vi "UMLEditor Main.vi"(1 "StartProject":string, 3 "StartTarget":string) -> ()   [LabVIEW 2020] (continued)
                        n383 = case shown="1.." w1168 {
                          tunnel: w1174 -> [w1175 w1184]
                          tunnel: [w1176 w1181] -> w1173
                          tunnel: [w1175 w1190] -> w1172
                          tunnel: w1171 -> [w1176 w1189]
                          tunnel: w1170 -> [_ w1188]
                          tunnel: w1169 -> [_ w1187]
                          tunnel: w1167 -> [_ w1183]
                          tunnel: w1166 -> [_ w1180]
                          frame 0, Default {
                          }
                          frame 1.. {
                            n384 = Index Array(array=w1187) -> (element=w1193:refnum<class "AbstractNode.lvclass">)  [unwired: 1 in]
                            n385 = Equal?(x=w1188, y=UMLEditor_HotSpotType."Collaps") -> (x = y?=w1194:bool)
                            n386 = call-dynamic "Collaps.vi"("reference in"=w1193, "Collaps"=w1194, "error in (no error)"=w1189) -> ("reference out"=w1179:refnum<class "AbstractNode.lvclass">, "error out"=w1192:errorcluster)  [unwired: 15 in]
                            n387 = Bundle By Name(cluster=w1184, "newSelected"=FALSE ("HotSpotCursor"), "state"=UMLEditor_statesType."Repaint", "lastMousePoint"=w1183) -> (w1185:T5)
                            n388 = Build Array(w1179) -> (w1178:refnum<class "AbstractNode.lvclass">[])
                            n389 = call <resource>:"UMLEditor setDiagramInfo.vi"("error in (no error)"=w1192, "localVariablesIn"=w1185, "action"=enum16{"Name/Dir", "Unsaved", "Saved"}."Unsaved") -> ("localVariablesOut"=w1190:T5, "error out"=w1182:errorcluster)  [unwired: 2 in, 13 out]
                            n390 = call-dynamic "layout.vi"("reference"=w1180, "LayoutNodes(Empty=All)"=w1178, "error in (no error)"=w1182) -> ("error out"=w1181:errorcluster)  [unwired: 15 in, 1 out]
                          }
                        }
                      }
                    }
                  }
                }
              }
              frame True {
              }
            }
            n391 = Bundle By Name(cluster=w899, "ShiftDown"=w880, "CtrlDown"=w880, "butDwn"=w880, "rubberBandStart"=w905, "dragStartPoint"=w905, "dragStartBounds"=T10 {"x"=nan, "y"=nan, "width"=nan, "height"=nan}) -> (w876:T5)
          }
          event "Picture": Mouse Wheel {
            n392 = event-data() -> ("Delta"=w1199:i32, "Orientation"=w1203:enum16{"Horizontal", "Vertical"}, "PlatMods"=w1205:T45)  [unwired: 3 out]
            n393 = Unbundle By Name(w1206) -> ("NodesBounds"=w1207:T10)
            n394 = Unbundle By Name(w1205) -> ("Ctrl"=w1204:bool)
            n395 = Multiply(x=w1199, y=25) -> (x*y=w1198:i32)
            n396 = disable-structure shown="Enabled" {
              disable-tunnel: [w1218 w1267] -> w1208
              disable-tunnel: w1207 -> [w1217 _]
              disable-tunnel: w1206 -> [w1216 w1267]
              disable-tunnel: w1204 -> [w1213 _]
              disable-tunnel: w1198 -> [w1212 _]
              disable-tunnel: w1203 -> [w1211 _]
              disable-tunnel: w1202 -> [w1210 w1266]
              disable-tunnel: [w1209 w1266] -> w1201
              frame Enabled {
                n397 = Unbundle By Name(w1217) -> ("height"=w1214:dbl, "width"=w1215:dbl)
                n398 = case shown="False" w1213 {
                  tunnel: w1212 -> [w1219 w1252]
                  tunnel: w1214 -> [w1245 _]
                  tunnel: w1216 -> [w1227 w1255]
                  tunnel: [w1227 w1256] -> w1218
                  tunnel: [w1239 w1254] -> w1209
                  tunnel: w1210 -> [w1239 w1253]
                  tunnel: w1215 -> [w1223 _]
                  tunnel: w1211 -> [_ _]
                  frame False {
                    w1231 = 0 ("lower limit")
                    n399 = Unbundle By Name(w1227) -> ("zoom"=w1224:dbl)
                    n400 = Multiply(x=w1224, y=w1245) -> (x*y=w1226:dbl)
                    n401 = Multiply(x=w1224, y=w1223) -> (x*y=w1225:dbl)
                    n402 = property on="Picture" class="Pict"() -> ("Draw Area Size"=w1248:T42)  [unwired: 2 in, 2 out]
                    n403 = To Long Integer(number=w1225) -> (32bit integer=w1235:i32)
                    n404 = To Long Integer(number=w1226) -> (32bit integer=w1242:i32)
                    n405 = property on="Picture" class="Pict"() -> ("Origin:Top"=w1221:i16, "Origin:Left"=w1230:i16)  [unwired: 2 in, 2 out]
                    n406 = Unbundle By Name(w1248) -> ("Height"=w1244:u32, "Width"=w1236:u32)
                    n407 = Subtract(x=w1221, y=w1219) -> (x-y=w1247:i32)
                    n408 = Subtract(x=w1230, y=w1219) -> (x-y=w1229:i32)
                    n409 = To Long Integer(number=w1236) -> (32bit integer=w1234:i32)
                    n410 = Subtract(x=w1235, y=w1234) -> (x-y=w1233:i32)
                    n411 = Max & Min(x=w1233, y=w1231) -> (max(x,y)=w1232:i32)  [unwired: 1 out]
                    n412 = In Range and Coerce(upper limit=w1232, x=w1229, lower limit=w1231) -> (coerced(x)=w1228:i32)  [unwired: 1 out]
                    n413 = To Long Integer(number=w1244) -> (32bit integer=w1237:i32)
                    n414 = Subtract(x=w1242, y=w1237) -> (x-y=w1243:i32)
                    n415 = Max & Min(x=w1243, y=0 ("lower limit")) -> (max(x,y)=w1240:i32)  [unwired: 1 out]
                    n416 = In Range and Coerce(upper limit=w1240, x=w1247, lower limit=0) -> (coerced(x)=w1222:i32)  [unwired: 1 out]
                    n417 = Not Equal?(x=w1222, y=w1221) -> (x != y?=w1220:bool)
                    n418 = Select(t=w1230, s=w1220, f=w1228) -> (s? t:f=w1238:i32)
                    n419 = property on="Picture" class="Pict"("Origin:Top"=w1222, "Origin:Left"=w1238) -> ()  [unwired: 2 in, 2 out]
                  }
                  frame True {
                    w1257 = 1.5 ("x")
                    n420 = Unbundle By Name(w1255) -> ("graphics"=w1264:refnum<class "Graphics.lvclass">, "zoom"=w1250:dbl)
                    n421 = Less Than 0?(x=w1252) -> (x < 0?=w1262:bool)
                    n422 = Not(x=w1262) -> (.not. x?=w1249:bool)
                    n423 = Multiply(x=w1250, y=w1257) -> (x*y=w1263:dbl)
                    n424 = Divide(x=w1250, y=w1257) -> (x/y=w1261:dbl)
                    n425 = Select(t=w1263, s=w1249, f=w1261) -> (s? t:f=w1260:dbl)
                    n426 = In Range and Coerce(upper limit=5.0625, x=w1260, lower limit=0.197530864) -> (coerced(x)=w1251:dbl)  [unwired: 1 out]
                    n427 = call <resource>:"scale.vi"("reference"=w1264, "scaleX"=w1251, "scaleY"=w1251, "error in (no error)"=w1253) -> ("error out"=w1254:errorcluster)  [unwired: 15 out]
                    n428 = Bundle By Name(cluster=w1255, "zoom"=w1251, "state"=UMLEditor_statesType."Repaint") -> (w1256:T5)
                  }
                }
              }
              frame Disabled {
              }
            }
          }
          event "Picture": Shortcut Menu Activation? {
            # "Show right click menus for graphs, node and edges"
            n429 = event-data() -> ("MenuRef"=w1291:refnum<k9>)  [unwired: 1 out]
            n430 = property on="Picture" class="Pict"() -> ("Mouse"=w1285:T41)  [unwired: 2 in, 2 out]
            n431 = Unbundle By Name(w1269) -> ("graphics"=w1273:refnum<class "Graphics.lvclass">)
            n432 = Delete Menu Items(6:w1290, 9:w1291) -> (0:w1278:errorcluster, 3:w1281:refnum<k9>)  [unwired: 2 out]
            n433 = Unbundle By Name(w1285) -> ("Mouse Position"=w1289:cluster{"X":i32, "Y":i32})
            n434 = Unbundle By Name(w1269) -> ("zoom"=w1286:dbl, "offset"=w1288:T9)
            n435 = Add(x=w1288, y=w1289) -> (x+y=w1287:T9)
            n436 = Divide(x=w1287, y=w1286) -> (x/y=w1270:T9)
            n437 = call <resource>:"UMLEditor_FindObject.vi"("offset"=w1270, "error in"=w1278, "graphics"=w1273, "graph"=w1275) -> ("error out"=w1271:errorcluster, "NodeFound"=w1277:bool, "node"=w1276:refnum<class "AbstractNode.lvclass">, "edge"=w1274:refnum<class "AbstractEdge.lvclass">, "EdgeFound"=w1272:bool)  [unwired: 2 in, 1 out]
            n438 = Bundle By Name(cluster=w1269, "lastMousePoint"=w1270) -> (w1268:T5)
            n439 = case shown="False" w1272 {
              tunnel: w1277 -> [w1308 _]
              tunnel: w1276 -> [w1307 _]
              tunnel: [w1306 w1339] -> w1280
              tunnel: w1268 -> [w1305 w1344]
              tunnel: [w1304 w1343] -> w1284
              tunnel: w1275 -> [w1303 _]
              tunnel: w1274 -> [_ w1345]
              tunnel: w1269 -> [w1302 _]
              tunnel: w1270 -> [w1301 _]
              tunnel: [w1300 w1340] -> w1282
              tunnel: w1271 -> [w1299 w1338]
              frame False {
                n440 = case shown="False" w1308 {
                  tunnel: w1307 -> [_ w1331]
                  tunnel: [w1313 w1323] -> w1306
                  tunnel: w1305 -> [w1319 w1329]
                  tunnel: [w1314 w1328] -> w1304
                  tunnel: w1303 -> [w1316 w1327]
                  tunnel: w1302 -> [_ _]
                  tunnel: w1301 -> [_ w1321]
                  tunnel: [w1312 w1324] -> w1300
                  tunnel: w1299 -> [w1310 w1322]
                  frame False {
                    n441 = call-dynamic "GetRightClickMenu.vi"("reference"=w1316, "error in (no error)"=w1310) -> ("Array"=w1312:string[], "error out"=w1313:errorcluster)  [unwired: 14 in, 2 out]
                    n442 = local write "GraphButtons"(T1."1" ("GraphButtons")) -> ()
                    n443 = Bundle By Name(cluster=w1319, "selected"=UMLEditor_tooltype."None" ("selcted"), "toolType"=UMLEditor_tooltype."None", "state"=UMLEditor_statesType."Repaint", "SelectedNodes"=refnum<class "AbstractNode.lvclass">[] [], "selectedEdge"=refnum<class "AbstractEdge.lvclass"> refnum) -> (w1314:T5)
                  }
                  frame True {
                    n444 = call-dynamic "GetNodeMenuOptions.vi"("reference"=w1331, "MousePos"=w1321, "error in (no error)"=w1322) -> ("reference out"=w1326:refnum<class "AbstractNode.lvclass">, "MenuOptions"=w1324:string[], "error out"=w1323:errorcluster)  [unwired: 14 in]
                    n445 = Array Size(array=w1324) -> (size(s)=w1330:i32)
                    n446 = Build Array(w1326) -> (w1325:refnum<class "AbstractNode.lvclass">[])
                    n447 = case shown="1.." w1330 {
                      tunnel: w1324 -> [_ _]
                      tunnel: w1329 -> [w1332 w1336]
                      tunnel: [w1332 w1335] -> w1328
                      tunnel: w1325 -> [_ w1334]
                      tunnel: w1327 -> [_ _]
                      frame 0, Default {
                      }
                      frame 1.. {
                        n448 = Bundle By Name(cluster=w1336, "selected"=UMLEditor_tooltype."Node" ("selcted"), "SelectedNodes"=w1334, "state"=UMLEditor_statesType."Repaint") -> (w1335:T5)
                      }
                    }
                  }
                }
              }
              frame True {
                n449 = call-dynamic "GetEdgeMenu.vi"("reference"=w1345, "error in (no error)"=w1338) -> ("reference out"=w1341:refnum<class "AbstractEdge.lvclass">, "MenuOptions"=w1340:string[], "error out"=w1339:errorcluster)  [unwired: 15 in]
                n450 = Array Size(array=w1340) -> (size(s)=w1342:i32)
                n451 = case shown="1.." w1342 {
                  tunnel: w1344 -> [w1346 w1350]
                  tunnel: [w1346 w1348] -> w1343
                  tunnel: w1341 -> [_ w1349]
                  frame 0, Default {
                  }
                  frame 1.. {
                    n452 = Bundle By Name(cluster=w1350, "selected"=UMLEditor_tooltype."Edge" ("selcted"), "selectedEdge"=w1349, "state"=UMLEditor_statesType."Repaint") -> (w1348:T5)
                  }
                }
              }
            }
            n453 = for {
              shift-right: [w1294] -> w1279
              shift-left: w1280 -> [w1296]
              tunnel: w1282 -> [w1295] mode=indexing
              tunnel: w1281 -> [w1292]
              n454 = case shown="Default" w1295 {
                selector: w1295 -> [w1297 _]
                tunnel: [w1297 "APP_SEPARATOR" ("after item")] -> w1293
                frame Default {
                }
                frame "" {
                }
              }
              n455 = Insert Menu Items(6:w1296, 7:w1293, 8:w1293, 9:w1292) -> (0:w1294:errorcluster)  [unwired: 4 out]
            }
            n456 = event-data("Discard?"=FALSE) -> ()  [unwired: 1 in, 1 out]
          }
          event "Picture": Shortcut Menu Selection (User) {
            n457 = event-data() -> ("ItemTag"=w1359:string)  [unwired: 1 out]
            n458 = Unbundle By Name(w1358) -> ("selected"=w1363:T7, "selectedEdge"=w1356:refnum<class "AbstractEdge.lvclass">, "SelectedNodes"=w1361:refnum<class "AbstractNode.lvclass">[])
            n459 = Unbundle By Name(w1354) -> ("graphics"=w1353:refnum<class "Graphics.lvclass">, "grid"=w1352:refnum<class "Grid.lvclass">)
            n460 = Index Array(array=w1361) -> (element=w1360:refnum<class "AbstractNode.lvclass">)  [unwired: 1 in]
            n461 = case shown="\"None\", Default" w1363 {
              tunnel: [w1371 w1405 w1454] -> w1364
              tunnel: [w1370 w1408 w1453] -> w1357
              tunnel: w1362 -> [w1369 w1411 w1450]
              tunnel: w1360 -> [_ _ w1452]
              tunnel: w1359 -> [w1368 w1409 w1451]
              tunnel: w1358 -> [w1366 w1407 w1449]
              tunnel: w1356 -> [w1367 _ _]
              tunnel: w1355 -> [w1365 w1410 w1448]
              tunnel: w1353 -> [_ _ w1447]
              tunnel: w1352 -> [_ _ w1446]
              frame "Edge" {
                n462 = case shown="Default" w1368 {
                  selector: w1368 -> [w1379 _ _]
                  tunnel: w1369 -> [w1381 w1398 w1402]
                  tunnel: w1366 -> [w1374 w1400 w1404]
                  tunnel: [w1376 w1397 w1401] -> w1370
                  tunnel: w1367 -> [w1380 _ _]
                  tunnel: [w1375 w1398 w1402] -> w1371
                  tunnel: w1365 -> [w1372 _ _]
                  frame Default {
                    n463 = call-dynamic "ExecuteMenuCommand.vi"("reference"=w1380, "Command"=w1379, "error in (no error)"=w1381) -> ("reference out"=w1377:refnum<class "AbstractEdge.lvclass">, "EditorAction"=w1378:T46, "error out"=w1373:errorcluster)  [unwired: 14 in]
                    n464 = case shown="\"ExecuteCommand\"" w1378 {
                      tunnel: w1374 -> [w1382 w1387 w1396]
                      tunnel: [w1382 w1386 w1393] -> w1376
                      tunnel: w1377 -> [_ _ _]
                      tunnel: w1373 -> [w1383 w1391 w1394]
                      tunnel: [w1383 w1389 w1394] -> w1375
                      tunnel: w1372 -> [_ w1385 _]
                      frame "NoAction", Default {
                      }
                      frame "Repaint" {
                        n465 = call-dynamic "layout.vi"("reference"=w1385, "error in (no error)"=w1391) -> ("error out"=w1390:errorcluster)  [unwired: 16 in, 1 out]
                        n466 = Bundle By Name(cluster=w1387, "state"=UMLEditor_statesType."Repaint") -> (w1384:T5)
                        n467 = call <resource>:"UMLEditor setDiagramInfo.vi"("error in (no error)"=w1390, "localVariablesIn"=w1384, "action"=enum16{"Name/Dir", "Unsaved", "Saved"}."Unsaved") -> ("localVariablesOut"=w1386:T5, "error out"=w1389:errorcluster)  [unwired: 2 in, 13 out]
                      }
                      frame "ExecuteCommand" {
                        n468 = Bundle By Name(cluster=w1396, "state"=UMLEditor_statesType."ExecuteCommand") -> (w1393:T5)
                      }
                    }
                  }
                  frame "Remove Edge" {
                    n469 = Bundle By Name(cluster=w1400, "state"=UMLEditor_statesType."RemoveSelected") -> (w1397:T5)
                  }
                  frame "Configure Edge" {
                    n470 = Bundle By Name(cluster=w1404, "state"=UMLEditor_statesType."EditSelected") -> (w1401:T5)
                  }
                }
              }
              frame "None", Default {
                n471 = Unbundle By Name(w1407) -> ("graphics"=w1414:refnum<class "Graphics.lvclass">, "grid"=w1413:refnum<class "Grid.lvclass">)
                n472 = Bundle By Name(cluster=w1407, "state"=UMLEditor_statesType."Repaint") -> (w1412:T5)
                n473 = case shown="Default" w1409 {
                  selector: w1409 -> [_ _ w1431]
                  tunnel: w1411 -> [w1417 w1418 w1438]
                  tunnel: [w1417 w1418 w1436] -> w1405
                  tunnel: w1414 -> [_ _ w1430]
                  tunnel: w1413 -> [_ _ w1429]
                  tunnel: w1412 -> [w1416 w1420 w1435]
                  tunnel: [w1416 w1419 w1434] -> w1408
                  tunnel: w1410 -> [_ _ w1432]
                  tunnel: w1407 -> [_ _ w1422]
                  frame "" {
                  }
                  frame "Apply Design Pattern..." {
                    n474 = Bundle By Name(cluster=w1420, "state"=UMLEditor_statesType."ApplyDesignPattern") -> (w1419:T5)
                  }
                  frame Default {
                    n475 = property on="Picture" class="Pict"() -> ("Mouse"=w1424:T41)  [unwired: 2 in, 2 out]
                    n476 = Unbundle By Name(w1424) -> ("Mouse Position"=w1428:cluster{"X":i32, "Y":i32})
                    n477 = Unbundle By Name(w1422) -> ("zoom"=w1425:dbl, "offset"=w1427:T9)
                    n478 = Add(x=w1427, y=w1428) -> (x+y=w1426:T9)
                    n479 = Divide(x=w1426, y=w1425) -> (x/y=w1423:T9)
                    n480 = call-dynamic "HandleRightClickMenuOption.vi"("reference"=w1432, "MenuOption"=w1431, "graphics"=w1430, "grid"=w1429, "point2D"=w1423, "error in (no error)"=w1438) -> ("Cancel"=w1433:bool, "error out"=w1437:errorcluster)  [unwired: 11 in, 1 out]
                    n481 = case shown="False" w1433 {
                      tunnel: w1437 -> [w1442 w1445]
                      tunnel: [w1441 w1445] -> w1436
                      tunnel: w1435 -> [w1439 w1444]
                      tunnel: [w1440 w1444] -> w1434
                      frame False {
                        n482 = call <resource>:"UMLEditor setDiagramInfo.vi"("error in (no error)"=w1442, "localVariablesIn"=w1439, "action"=enum16{"Name/Dir", "Unsaved", "Saved"}."Unsaved") -> ("localVariablesOut"=w1440:T5, "error out"=w1441:errorcluster)  [unwired: 2 in, 13 out]
                      }
                      frame True {
                      }
                    }
                  }
                }
                n483 = local write "GraphButtons"(T1."1" ("GraphButtons")) -> ()
              }
              frame "Node" {
                n484 = case shown="Default" w1451 {
                  selector: w1451 -> [w1462 _ w1487 _ _]
                  tunnel: w1450 -> [w1464 w1484 w1491 w1523 w1532]
                  tunnel: w1449 -> [w1457 w1482 w1486 w1521 w1534]
                  tunnel: [w1459 w1481 w1485 w1520 w1531] -> w1453
                  tunnel: w1452 -> [w1463 _ _ w1516 _]
                  tunnel: [w1458 w1484 w1491 w1522 w1532] -> w1454
                  tunnel: w1448 -> [w1455 _ _ w1519 _]
                  tunnel: w1447 -> [_ _ _ w1518 _]
                  tunnel: w1446 -> [_ _ _ w1517 _]
                  frame Default {
                    n485 = call-dynamic "ExecuteMenuCommand.vi"("reference"=w1463, "Command"=w1462, "error in (no error)"=w1464) -> ("EditorAction"=w1461:T46, "FlattenCommandSettings"=w1460:T12, "error out"=w1456:errorcluster)  [unwired: 13 in, 1 out]
                    n486 = case shown="\"ExecuteCommand\"" w1461 {
                      tunnel: w1457 -> [w1465 w1469 w1480]
                      tunnel: [w1465 w1470 w1476] -> w1459
                      tunnel: w1460 -> [_ _ w1478]
                      tunnel: w1456 -> [w1466 w1474 w1477]
                      tunnel: [w1466 w1472 w1477] -> w1458
                      tunnel: w1455 -> [_ w1467 _]
                      frame "NoAction", Default {
                      }
                      frame "Repaint" {
                        n487 = call-dynamic "layout.vi"("reference"=w1467, "error in (no error)"=w1474) -> ("error out"=w1473:errorcluster)  [unwired: 16 in, 1 out]
                        n488 = Bundle By Name(cluster=w1469, "state"=UMLEditor_statesType."Repaint") -> (w1468:T5)
                        n489 = call <resource>:"UMLEditor setDiagramInfo.vi"("error in (no error)"=w1473, "localVariablesIn"=w1468, "action"=enum16{"Name/Dir", "Unsaved", "Saved"}."Unsaved") -> ("localVariablesOut"=w1470:T5, "error out"=w1472:errorcluster)  [unwired: 2 in, 13 out]
                      }
                      frame "ExecuteCommand" {
                        n490 = Bundle By Name(cluster=w1480, "state"=UMLEditor_statesType."ExecuteCommand", "FlattenCommandSettings"=w1478) -> (w1476:T5)
                      }
                    }
                  }
                  frame "Apply Design Pattern..." {
                    n491 = Bundle By Name(cluster=w1482, "state"=UMLEditor_statesType."ApplyDesignPattern") -> (w1481:T5)
                  }
                  frame "Remove Node", "Remove package only" {
                    n492 = Equal?(x=w1487, y="Remove package only") -> (x = y?=w1488:bool)
                    n493 = Bundle By Name(cluster=w1486, "state"=UMLEditor_statesType."RemoveSelected", "Don'tDeleteChildren"=w1488) -> (w1485:T5)
                  }
                  frame "Disconnect from package" {
                    n494 = call-dynamic "GetParentsRecurivly.vi"("reference"=w1516, "error in (no error)"=w1523) -> ("Parents"=w1494:refnum<class "AbstractNode.lvclass">[], "error out"=w1496:errorcluster)  [unwired: 15 in, 1 out]
                    n495 = Index Array(array=w1494) -> (element=w1493:refnum<class "AbstractNode.lvclass">)  [unwired: 1 in]
                    n496 = call-dynamic "removeChild.vi"("reference"=w1493, "node"=w1516, "error in (no error)"=w1496) -> ("reference out"=w1509:refnum<class "AbstractNode.lvclass">, "error out"=w1512:errorcluster)  [unwired: 15 in]
                    n497 = call-dynamic "setParent.vi"("reference"=w1516, "node"=refnum<class "AbstractNode.lvclass"> refnum, "error in (no error)"=w1512) -> ("error out"=w1510:errorcluster)  [unwired: 15 in, 1 out]
                    n498 = call-dynamic "layout.vi"("reference"=w1509, "graph"=w1519, "graphics"=w1518, "grid"=w1517, "error in (no error)"=w1510) -> ("error out"=w1508:errorcluster)  [unwired: 13 in, 1 out]
                    n499 = Delete From Array(array=w1494) -> (deleted portion=w1495:refnum<class "AbstractNode.lvclass">)  [unwired: 2 in, 1 out]
                    n500 = call-dynamic "getBounds.vi"("reference"=w1495, "error in (no error)"=w1508) -> ("bounds"=w1506:T10, "error out"=w1507:errorcluster)  [unwired: 15 in, 1 out]
                    n501 = call <resource>:"Rectangel GetRectInfo.vi"("bounds"=w1506) -> ("maxX"=w1504:dbl)  [unwired: 1 in, 17 out]
                    n502 = call-dynamic "getBounds.vi"("reference"=w1516, "error in (no error)"=w1507) -> ("reference out"=w1499:refnum<class "AbstractNode.lvclass">, "bounds"=w1505:T10, "error out"=w1498:errorcluster)  [unwired: 15 in]
                    n503 = Unbundle By Name(w1505) -> ("x"=w1503:dbl)
                    n504 = Subtract(x=w1504, y=w1503) -> (x-y=w1502:dbl)
                    n505 = Add(x=10.0, y=w1502) -> (x+y=w1500:dbl)
                    n506 = Greater Or Equal To 0?(x=w1500) -> (x >= 0?=w1497:bool)
                    n507 = case shown="True" w1497 {
                      tunnel: [w1525 w1530] -> w1515
                      tunnel: w1500 -> [_ w1529]
                      tunnel: w1499 -> [_ w1528]
                      tunnel: w1498 -> [w1525 w1527]
                      frame False {
                      }
                      frame True {
                        n508 = call-dynamic "translate.vi"("reference"=w1528, "dx"=w1529, "dy"=0.0, "error in (no error)"=w1527) -> ("error out"=w1530:errorcluster)  [unwired: 14 in, 1 out]
                      }
                    }
                    n509 = Bundle By Name(cluster=w1521, "state"=UMLEditor_statesType."Repaint") -> (w1492:T5)
                    n510 = call-dynamic "layout.vi"("reference"=w1519, "error in (no error)"=w1515) -> ("error out"=w1513:errorcluster)  [unwired: 16 in, 1 out]
                    n511 = call <resource>:"UMLEditor setDiagramInfo.vi"("error in (no error)"=w1513, "localVariablesIn"=w1492, "action"=enum16{"Name/Dir", "Unsaved", "Saved"}."Unsaved") -> ("localVariablesOut"=w1520:T5, "error out"=w1522:errorcluster)  [unwired: 2 in, 13 out]
                  }
                  frame "Configure Node" {
                    n512 = Bundle By Name(cluster=w1534, "state"=UMLEditor_statesType."EditSelected") -> (w1531:T5)
                  }
                }
              }
            }
          }
          event "PictureMenuEvent": Value Change {
            n513 = event-data() -> ("NewVal"=w1535:string)  [unwired: 1 out]
            n514 = Unbundle By Name(w1539) -> ("selected"=w1543:T7, "selectedEdge"=w1537:refnum<class "AbstractEdge.lvclass">, "SelectedNodes"=w1541:refnum<class "AbstractNode.lvclass">[])
            n515 = Index Array(array=w1541) -> (element=w1540:refnum<class "AbstractNode.lvclass">)  [unwired: 1 in]
            n516 = case shown="\"None\", Default" w1543 {
              tunnel: [w1551 w1586 w1628] -> w1544
              tunnel: [w1550 w1588 w1627] -> w1538
              tunnel: w1542 -> [w1549 w1591 w1624]
              tunnel: w1540 -> [_ _ w1626]
              tunnel: w1535 -> [w1548 w1589 w1625]
              tunnel: w1539 -> [w1546 w1587 w1623]
              tunnel: w1537 -> [w1547 _ _]
              tunnel: w1536 -> [w1545 w1590 w1622]
              frame "Edge" {
                n517 = case shown="Default" w1548 {
                  selector: w1548 -> [w1559 _ _]
                  tunnel: w1549 -> [w1561 w1578 w1582]
                  tunnel: w1546 -> [w1554 w1580 w1584]
                  tunnel: [w1556 w1577 w1581] -> w1550
                  tunnel: w1547 -> [w1560 _ _]
                  tunnel: [w1555 w1578 w1582] -> w1551
                  tunnel: w1545 -> [w1552 _ _]
                  frame Default {
                    n518 = call-dynamic "ExecuteMenuCommand.vi"("reference"=w1560, "Command"=w1559, "error in (no error)"=w1561) -> ("reference out"=w1557:refnum<class "AbstractEdge.lvclass">, "EditorAction"=w1558:T46, "error out"=w1553:errorcluster)  [unwired: 14 in]
                    n519 = case shown="\"ExecuteCommand\"" w1558 {
                      tunnel: w1554 -> [w1562 w1567 w1576]
                      tunnel: [w1562 w1566 w1573] -> w1556
                      tunnel: w1557 -> [_ _ _]
                      tunnel: w1553 -> [w1563 w1571 w1574]
                      tunnel: [w1563 w1569 w1574] -> w1555
                      tunnel: w1552 -> [_ w1565 _]
                      frame "NoAction", Default {
                      }
                      frame "Repaint" {
                        n520 = call-dynamic "layout.vi"("reference"=w1565, "error in (no error)"=w1571) -> ("error out"=w1570:errorcluster)  [unwired: 16 in, 1 out]
                        n521 = Bundle By Name(cluster=w1567, "state"=UMLEditor_statesType."Repaint") -> (w1564:T5)
                        n522 = call <resource>:"UMLEditor setDiagramInfo.vi"("error in (no error)"=w1570, "localVariablesIn"=w1564, "action"=enum16{"Name/Dir", "Unsaved", "Saved"}."Unsaved") -> ("localVariablesOut"=w1566:T5, "error out"=w1569:errorcluster)  [unwired: 2 in, 13 out]
                      }
                      frame "ExecuteCommand" {
                        n523 = Bundle By Name(cluster=w1576, "state"=UMLEditor_statesType."ExecuteCommand") -> (w1573:T5)
                      }
                    }
                  }
                  frame "Remove Edge" {
                    n524 = Bundle By Name(cluster=w1580, "state"=UMLEditor_statesType."RemoveSelected") -> (w1577:T5)
                  }
                  frame "Configure Edge" {
                    n525 = Bundle By Name(cluster=w1584, "state"=UMLEditor_statesType."EditSelected") -> (w1581:T5)
                  }
                }
              }
              frame "None", Default {
                n526 = Unbundle By Name(w1587) -> ("graphics"=w1594:refnum<class "Graphics.lvclass">, "grid"=w1593:refnum<class "Grid.lvclass">)
                n527 = Bundle By Name(cluster=w1587, "state"=UMLEditor_statesType."Repaint") -> (w1592:T5)
                n528 = case shown="Default" w1589 {
                  selector: w1589 -> [_ w1607]
                  tunnel: w1591 -> [w1597 w1614]
                  tunnel: [w1597 w1612] -> w1586
                  tunnel: w1594 -> [_ w1606]
                  tunnel: w1593 -> [_ w1605]
                  tunnel: w1592 -> [w1596 w1611]
                  tunnel: [w1596 w1610] -> w1588
                  tunnel: w1590 -> [_ w1608]
                  tunnel: w1587 -> [_ w1598]
                  frame "" {
                  }
                  frame Default {
                    n529 = property on="Picture" class="Pict"() -> ("Mouse"=w1600:T41)  [unwired: 2 in, 2 out]
                    n530 = Unbundle By Name(w1600) -> ("Mouse Position"=w1604:cluster{"X":i32, "Y":i32})
                    n531 = Unbundle By Name(w1598) -> ("zoom"=w1601:dbl, "offset"=w1603:T9)
                    n532 = Add(x=w1603, y=w1604) -> (x+y=w1602:T9)
                    n533 = Divide(x=w1602, y=w1601) -> (x/y=w1599:T9)
                    n534 = call-dynamic "HandleRightClickMenuOption.vi"("reference"=w1608, "MenuOption"=w1607, "graphics"=w1606, "grid"=w1605, "point2D"=w1599, "error in (no error)"=w1614) -> ("Cancel"=w1609:bool, "error out"=w1613:errorcluster)  [unwired: 11 in, 1 out]
                    n535 = case shown="False" w1609 {
                      tunnel: w1613 -> [w1618 w1621]
                      tunnel: [w1617 w1621] -> w1612
                      tunnel: w1611 -> [w1615 w1620]
                      tunnel: [w1616 w1620] -> w1610
                      frame False {
                        n536 = call <resource>:"UMLEditor setDiagramInfo.vi"("error in (no error)"=w1618, "localVariablesIn"=w1615, "action"=enum16{"Name/Dir", "Unsaved", "Saved"}."Unsaved") -> ("localVariablesOut"=w1616:T5, "error out"=w1617:errorcluster)  [unwired: 2 in, 13 out]
                      }
                      frame True {
                      }
                    }
                  }
                }
                n537 = local write "GraphButtons"(T1."1" ("GraphButtons")) -> ()
              }
              frame "Node" {
                n538 = case shown="Default" w1625 {
                  selector: w1625 -> [w1636 _ _]
                  tunnel: w1624 -> [w1638 w1656 w1660]
                  tunnel: w1623 -> [w1631 w1658 w1662]
                  tunnel: [w1633 w1655 w1659] -> w1627
                  tunnel: w1626 -> [w1637 _ _]
                  tunnel: [w1632 w1656 w1660] -> w1628
                  tunnel: w1622 -> [w1629 _ _]
                  frame Default {
                    n539 = call-dynamic "ExecuteMenuCommand.vi"("reference"=w1637, "Command"=w1636, "error in (no error)"=w1638) -> ("EditorAction"=w1635:T46, "FlattenCommandSettings"=w1634:T12, "error out"=w1630:errorcluster)  [unwired: 13 in, 1 out]
                    n540 = case shown="\"ExecuteCommand\"" w1635 {
                      tunnel: w1631 -> [w1639 w1643 w1654]
                      tunnel: [w1639 w1644 w1650] -> w1633
                      tunnel: w1634 -> [_ _ w1652]
                      tunnel: w1630 -> [w1640 w1648 w1651]
                      tunnel: [w1640 w1646 w1651] -> w1632
                      tunnel: w1629 -> [_ w1641 _]
                      frame "NoAction", Default {
                      }
                      frame "Repaint" {
                        n541 = call-dynamic "layout.vi"("reference"=w1641, "error in (no error)"=w1648) -> ("error out"=w1647:errorcluster)  [unwired: 16 in, 1 out]
                        n542 = Bundle By Name(cluster=w1643, "state"=UMLEditor_statesType."Repaint") -> (w1642:T5)
                        n543 = call <resource>:"UMLEditor setDiagramInfo.vi"("error in (no error)"=w1647, "localVariablesIn"=w1642, "action"=enum16{"Name/Dir", "Unsaved", "Saved"}."Unsaved") -> ("localVariablesOut"=w1644:T5, "error out"=w1646:errorcluster)  [unwired: 2 in, 13 out]
                      }
                      frame "ExecuteCommand" {
                        n544 = Bundle By Name(cluster=w1654, "state"=UMLEditor_statesType."ExecuteCommand", "FlattenCommandSettings"=w1652) -> (w1650:T5)
                      }
                    }
                  }
                  frame "Remove Node" {
                    n545 = Bundle By Name(cluster=w1658, "state"=UMLEditor_statesType."RemoveSelected") -> (w1655:T5)
                  }
                  frame "Configure Node" {
                    n546 = Bundle By Name(cluster=w1662, "state"=UMLEditor_statesType."EditSelected") -> (w1659:T5)
                  }
                }
              }
            }
          }
          event "Project": Mouse Down? {
            n547 = event-data() -> ()  [unwired: 2 out]
            n548 = property on="Project" class="Ring (strict)"() -> ("Strings []"=w1664:string[])  [unwired: 2 in, 2 out]
            n549 = call <resource>:"UMLEditor getDiagramInfo.vi"("localVariables"=w1673, "error in (no error)"=w1671) -> ("graph"=w1670:refnum<class "Graph.lvclass">, "error out"=w1669:errorcluster)  [unwired: 16 out]
            n550 = Index Array(array=w1664) -> (element=w1666:string)  [unwired: 1 in]
            n551 = Empty String/Path?(string/path=w1666) -> (empty?=w1665:bool)
            n552 = call-dynamic "getNodes.vi"("reference"=w1670, "error in (no error)"=w1669) -> ("nodes"=w1668:refnum<class "AbstractNode.lvclass">[])  [unwired: 15 in, 2 out]
            n553 = Empty Array?(array=w1668) -> (empty?=w1667:bool)
            n554 = Or(x=w1667, y=w1665) -> ()  [unwired: 1 out]
            n555 = case shown="True" TRUE {
              tunnel: w1671 -> [w1676 w1685]
              tunnel: [w1676 w1684] -> w1674
              tunnel: [TRUE ("Discard?") w1683] -> w1672
              tunnel: w1664 -> [_ w1680]
              frame False {
                n556 = One Button Dialog(message="You are only allowed to change project if the current diagram is empty.") -> ()  [unwired: 2 out]
              }
              frame True {
                n557 = call <resource>:"GDSProject_GetProjects.vi"("error in (no error)"=w1685, "OpenProjectRef(True)"=FALSE) -> ("Projects"=w1679:string[], "error out"=w1684:errorcluster)  [unwired: 1 in, 15 out]
                n558 = Index Array(array=w1679) -> (element=w1682:string)  [unwired: 1 in]
                n559 = Empty String/Path?(string/path=w1682) -> (empty?=w1681:bool)
                n560 = case shown="True" w1681 {
                  tunnel: [FALSE ("Discard?") TRUE ("Discard?")] -> w1683
                  tunnel: w1679 -> [w1688 _]
                  tunnel: w1680 -> [w1687 _]
                  frame False {
                    n561 = for {
                      tunnel: w1688 -> [w1690] mode=indexing
                      shift-right: [w1693] -> w1686
                      shift-left: w1687 -> [w1692]
                      n562 = Search 1D Array(1D array=w1692, element=w1690) -> (index of element=w1691:i32)  [unwired: 1 out]
                      n563 = case shown="0, Default" w1691 {
                        tunnel: [w1694 w1697] -> w1693
                        tunnel: w1692 -> [w1694 w1696]
                        tunnel: w1690 -> [_ w1695]
                        frame 0, Default {
                        }
                        frame -1 {
                          n564 = Build Array (concatenate)(w1696, w1695) -> (w1697:string[])
                        }
                      }
                    }
                    n565 = property on="Project" class="Ring (strict)"("Strings []"=w1686) -> ()  [unwired: 2 in, 2 out]
                  }
                  frame True {
                    n566 = call "File Dialog"("prompt"="Select a project to open", "button label"="Open", "pattern (all files)"="*.lvproj", "pattern label"="LabVIEW projects") -> ("selected path"=w1698:path, "cancelled"=w1699:bool)  [unwired: 3 in, 7 out]
                    n567 = case shown="False" w1699 {
                      tunnel: w1698 -> [w1721 _]
                      frame False {
                        n568 = call <vilib>:"Set Busy.vi"() -> ("error out"=w1715:errorcluster)  [unwired: 4 in, 7 out]
                        n569 = call <vilib>:"Clear Errors.vi"("error in (no error)"=w1715) -> ("error out"=w1705:errorcluster)  [unwired: 5 in, 1 out]
                        n570 = call <resource>:"GetRelativePathOption.vi"() -> ("UseProjectFolderAsBasePath"=w1708:bool)  [unwired: 1 in, 18 out]
                        n571 = invoke class="App" method="Project.Open"(error in=w1705, "Path"=w1721) -> ("Project:Open"=w1720:refnum<vi>)  [unwired: 2 in, 3 out]
                        n572 = invoke class="Project" method="Open Window"(reference=w1720) -> (reference out=w1718:refnum<vi>, error out=w1719:errorcluster)  [unwired: 2 in, 1 out]
                        n573 = Close Reference(reference=w1718, error in (no error)=w1719) -> (error out=w1717:errorcluster)
                        n574 = call <resource>:"GDSProject_GetProjects.vi"("error in (no error)"=w1717, "OpenProjectRef(True)"=FALSE) -> ("Projects"=w1716:string[])  [unwired: 1 in, 16 out]
                        n575 = Index Array(array=w1716) -> (element=w1713:string)  [unwired: 1 in]
                        n576 = call <resource>:"UMLEditor_TargetDialog.vi"("GetProjectRefByName"=w1713) -> ("error out"=w1712:errorcluster, "ProjectFolder"=w1706:path, "TargetIndex"=w1710:u16, "Targets"=w1711:string[])  [unwired: 6 in, 1 out]
                        n577 = case shown="True" w1708 {
                          tunnel: w1706 -> [_ w1723]
                          tunnel: File_StoredPathesActions."Set Path" ("Method (Get Path)") -> [_ w1722]
                          frame False {
                          }
                          frame True {
                            n578 = call <resource>:"File_ApplicationPaths.vi"("PathName"=UMLEditor_StoredPathes."ClassBasePath" ("UMLPathes"), "Path In"=w1723, "Method (Get Path)"=w1722) -> ()  [unwired: 1 in, 16 out]
                          }
                        }
                        n579 = property on="Target" class="Ring (strict)"("Strings []"=w1711, "Value"=w1710) -> ()  [unwired: 2 in, 2 out]
                        n580 = Build Array(w1713) -> (w1714:string[])
                        n581 = property on="Project" class="Ring (strict)"("Strings []"=w1714) -> ()  [unwired: 2 in, 2 out]
                        n582 = call <vilib>:"Unset Busy.vi"("error in (no error)"=w1712) -> ()  [unwired: 1 in, 10 out]
                      }
                      frame True {
                      }
                    }
                  }
                }
              }
            }
            n583 = event-data("Discard?"=w1672) -> ()  [unwired: 1 in, 1 out]
          }
          event "Project": Value Change {
            n584 = event-data() -> ()  [unwired: 2 out]
            n585 = property on="Project" class="Ring (strict)"() -> ("Strings []"=w1736:string[])  [unwired: 2 in, 2 out]
            n586 = Index Array(array=w1736, index="Project") -> (element=w1729:string)
            n587 = call <resource>:"UMLEditor_TargetDialog.vi"("error in (no error)"=w1730, "GetProjectRefByName"=w1729) -> ("error out"=w1727:errorcluster, "ProjectFolder"=w1728:path, "TargetIndex"=w1726:u16, "Targets"=w1725:string[])  [unwired: 5 in, 1 out]
            n588 = call <resource>:"GetRelativePathOption.vi"() -> ("UseProjectFolderAsBasePath"=w1734:bool)  [unwired: 1 in, 18 out]
            n589 = property on="Target" class="Ring (strict)"("Strings []"=w1725, "Value"=w1726) -> ()  [unwired: 2 in, 2 out]
            n590 = case shown="True" w1734 {
              tunnel: w1728 -> [_ w1756]
              tunnel: File_StoredPathesActions."Set Path" ("Method (Get Path)") -> [_ w1755]
              frame False {
              }
              frame True {
                n591 = call <resource>:"File_ApplicationPaths.vi"("PathName"=UMLEditor_StoredPathes."ClassBasePath" ("UMLPathes"), "Path In"=w1756, "Method (Get Path)"=w1755) -> ()  [unwired: 1 in, 16 out]
              }
            }
            n592 = Unbundle By Name(w1727) -> ("code"=w1732:i32)
            n593 = case shown="1055" w1732 {
              tunnel: w1727 -> [w1738 _]
              tunnel: [w1738 w1747] -> w1731
              tunnel: w1730 -> [_ w1747]
              frame 0, Default {
              }
              frame 1055 {
                n594 = call <resource>:"GDSProject_GetProjects.vi"("OpenProjectRef(True)"=FALSE) -> ("Projects"=w1748:string[])  [unwired: 2 in, 16 out]
                n595 = Index Array(array=w1748) -> (element=w1746:string)  [unwired: 1 in]
                n596 = stacked-sequence {
                  tunnel: [w1753] -> w1745
                  tunnel: w1746 -> [w1753]
                  frame #0 {
                    n597 = One Button Dialog(message="The selected project has been closed.\nSelect another one.") -> ()  [unwired: 2 out]
                  }
                }
                n598 = call <resource>:"UMLEditor_TargetDialog.vi"("GetProjectRefByName"=w1745) -> ("ProjectFolder"=w1739:path, "TargetIndex"=w1744:u16, "Targets"=w1743:string[])  [unwired: 6 in, 2 out]
                n599 = call <resource>:"GetRelativePathOption.vi"() -> ("UseProjectFolderAsBasePath"=w1741:bool)  [unwired: 1 in, 18 out]
                n600 = case shown="True" w1741 {
                  tunnel: w1739 -> [_ w1751]
                  tunnel: File_StoredPathesActions."Set Path" ("Method (Get Path)") -> [_ w1750]
                  frame False {
                  }
                  frame True {
                    n601 = call <resource>:"File_ApplicationPaths.vi"("PathName"=UMLEditor_StoredPathes."ClassBasePath" ("UMLPathes"), "Path In"=w1751, "Method (Get Path)"=w1750) -> ()  [unwired: 1 in, 16 out]
                  }
                }
                n602 = property on="Project" class="Ring (strict)"("Strings []"=w1748, "Value"=0) -> ()  [unwired: 2 in, 2 out]
                n603 = property on="Target" class="Ring (strict)"("Strings []"=w1743, "Value"=w1744) -> ()  [unwired: 2 in, 2 out]
              }
            }
          }
          event "RevHistory": Mouse Down {
            n604 = event-data() -> ("Mods.Double Click"=w1758:bool)  [unwired: 1 out]
            n605 = case shown="True" w1758 {
              tunnel: w1761 -> [w1762 w1765]
              tunnel: [w1762 w1764] -> w1760
              tunnel: w1759 -> [_ w1763]
              frame False {
              }
              frame True {
                n606 = call <resource>:"UMLEditor RevisionHistory.vi"("localVariables"=w1763, "error in (no error)"=w1765) -> ("error out"=w1764:errorcluster)  [unwired: 17 out]
              }
            }
          }
          event "Sync": Value Change {
            n607 = event-data() -> ()  [unwired: 2 out]
            n608 = case shown="True" "Sync" {
              selector: "Sync" -> [_ w1773]
              tunnel: [FALSE w1775] -> w1766
              tunnel: w1768 -> [_ w1774]
              frame False {
                n609 = local write "StatusBar"("" ("StatusBar")) -> ()
              }
              frame True {
                n610 = call <resource>:"UMLEditor getDiagramInfo.vi"("localVariables"=w1774) -> ("graph"=w1776:refnum<class "Graph.lvclass">, "diagramType"=w1777:T27)  [unwired: 1 in, 16 out]
                n611 = case shown="\"ClassDiagramGraph\"" w1777 {
                  tunnel: w1773 -> [_ _]
                  tunnel: w1776 -> [_ w1790]
                  tunnel: [FALSE w1789] -> w1775
                  frame "None", Default {
                    n612 = One Button Dialog(message="Only class diagrams can have auto synchronization turn on.") -> ()  [unwired: 1 in, 1 out]
                  }
                  frame "ClassDiagramGraph" {
                    n613 = call-dynamic "getNodes.vi"("reference"=w1790) -> ("nodes"=w1788:refnum<class "AbstractNode.lvclass">[])  [unwired: 16 in, 2 out]
                    n614 = call <resource>:"CommonVIs_UmlOpenVIRef.vi"() -> ("AppRefOut"=w1783:refnum<vi>)  [unwired: 4 in, 7 out]
                    n615 = property class="App"(reference=w1783) -> ("App.AllMyLibses"=w1782:string[])  [unwired: 1 in, 2 out]
                    n616 = Array Size(array=w1788) -> (size(s)=w1787:i32)
                    n617 = Equal To 0?(x=w1787) -> (x = 0?=w1786:bool)
                    n618 = for {
                      tunnel: w1782 -> [w1794] mode=indexing
                      tunnel: [w1791] -> w1781 mode=indexing
                      n619 = call <resource>:"GDSString_FindWord.vi"("Text"=w1794, "PatternMatchingDelimiter(\\s\\t\\r\\n)"=":" ("PatternMatchingDelimiter(\\s\\t\\r\\n)"), "Search Backwards"=TRUE) -> ("NextWord"=w1791:string)  [unwired: 11 in, 5 out]
                    }
                    n620 = To Lower Case(string=w1781) -> (all lower case string=w1780:string[])
                    n621 = for {
                      tunnel: w1788 -> [w1802] mode=indexing
                      tunnel: [w1798] -> w1784
                      tunnel: w1780 -> [w1797]
                      stop <- w1798 continue-if-true
                      w1801 = refnum<class "ClassNode.lvclass"> refnum  # ClassNode.lvclass
                      n622 = To More Specific Class(target class=w1801, reference=w1802) -> (specific class reference=w1800:refnum<class "ClassNode.lvclass">, error out=w1799:errorcluster)  [unwired: 1 in]
                      n623 = case shown="No Error" w1799 {
                        selector: w1799 -> [w1809 _]
                        tunnel: w1800 -> [w1810 _]
                        tunnel: [w1803 TRUE] -> w1798
                        tunnel: w1797 -> [w1805 _]
                        frame No Error {
                          n624 = call-dynamic "getClassInfo.vi"("reference"=w1810, "error in (no error)"=w1809) -> ("ClassPath"=w1808:path)  [unwired: 8 in, 9 out]
                          n625 = Strip Path(path=w1808) -> (name=w1807:string)  [unwired: 1 out]
                          n626 = To Lower Case(string=w1807) -> (all lower case string=w1806:string)
                          n627 = Search 1D Array(1D array=w1805, element=w1806) -> (index of element=w1804:i32)  [unwired: 1 in]
                          n628 = Less Than 0?(x=w1804) -> (x < 0?=w1803:bool)
                        }
                        frame Error {
                        }
                      }
                    }
                    n629 = Or(x=w1784, y=w1786) -> (x .or. y?=w1785:bool)
                    n630 = case shown="True" w1785 {
                      tunnel: [TRUE _] -> w1789
                      frame False {
                      }
                      frame True {
                        n631 = One Button Dialog(message="Synchronization can't be turned on for this diagram. Make sure at least one class have a class path defined and that the classes are in memory.") -> ()  [unwired: 1 in, 1 out]
                      }
                    }
                  }
                }
              }
            }
            n632 = Bundle By Name(cluster=w1768, "ForceSyncNow"=w1766, "Sync"=w1766) -> (w1769:T5)
            n633 = local write "Sync"(w1766) -> ()
          }
          event "Target": Value Change {
            n634 = event-data() -> ()  [unwired: 7 out]
            n635 = property on="Target" class="Ring (strict)"() -> ("Strings []"=w1820:string[], "Value"=w1819:u16)  [unwired: 2 in, 2 out]
            n636 = property on="Project" class="Ring (strict)"() -> ("Strings []"=w1815:string[], "Value"=w1814:u16)  [unwired: 2 in, 2 out]
            n637 = Index Array(array=w1820, index=w1819) -> (element=w1818:string)
            n638 = Index Array(array=w1815, index=w1814) -> (element=w1813:string)
            n639 = call <resource>:"UMLEditor_TargetDialog.vi"("error in (no error)"=w1817, "Target"=w1818, "GetProjectRefByName"=w1813) -> ("error out"=w1816:errorcluster)  [unwired: 4 in, 4 out]
          }
          event Mouse Enter {
            n640 = event-data() -> ("CtlRef"=w1822:refnum<vi>)  [unwired: 1 out]
            n641 = Unbundle By Name(w1826) -> ("ToolHelp"=w1828:bool)
            n642 = local read "Help"() -> (w1827:bool)
            n643 = And(x=w1828, y=w1827) -> (x .and. y?=w1825:bool)
            n644 = case shown="True" w1825 {
              tunnel: w1824 -> [w1829 w1834]
              tunnel: [w1829 w1839] -> w1823
              tunnel: w1822 -> [_ w1838]
              tunnel: w1821 -> [_ w1832]
              frame False {
              }
              frame True {
                w1836 = refnum<vi> refnum  # Boolean
                n645 = To More Specific Class(target class=w1836, reference=w1838) -> (specific class reference=w1837:refnum<vi>)  [unwired: 1 in, 1 out]
                n646 = property class="Bool"(reference=w1837) -> ("Strings [4]"=w1835:string[])  [unwired: 1 in, 2 out]
                n647 = Index Array(array=w1835) -> (element=w1831:string)  [unwired: 1 in]
                n648 = call-dynamic "GetButtonHelpText.vi"("reference in"=w1832, "ButtonString"=w1831, "error in (no error)"=w1834) -> ("HelpOut"=w1830:T38, "error out"=w1833:errorcluster)  [unwired: 14 in, 1 out]
                n649 = call <resource>:"ContextHelp_SendMessageToPopUp.vi"("PopUpMessage"=w1830, "error in (no error)"=w1833) -> ("error out"=w1839:errorcluster)  [unwired: 1 in, 16 out]
              }
            }
          }
          event User Event {
            # "WholeProject"
            # "ReverseEngineering:Class:%s:%s"
            n650 = event-data() -> ("Action"=w1841:string, "Data"=w1840:string)  [unwired: 1 out]
            n651 = case shown="\"ReverseEngineering\"" w1841 {
              tunnel: w1845 -> [w1847 w1871 w1924 w1945]
              tunnel: [w1847 w1870 w1923 w1944] -> w1844
              tunnel: w1840 -> [_ w1869 w1922 w1946]
              tunnel: w1843 -> [w1846 w1867 w1920 w1942]
              tunnel: [w1846 w1866 w1919 w1942] -> w1842
              frame "False", Default {
              }
              frame "ReverseEngineering" {
                n652 = Match Pattern(string=w1869, regular expression=":") -> (before substring=w1856:string, after substring=w1864:string)  [unwired: 3 out]
                n653 = Match Pattern(string=w1864, regular expression=":") -> (before substring=w1863:string, after substring=w1854:string)  [unwired: 3 out]
                n654 = Reverse String(1:w1854) -> (0:w1853:string)
                n655 = Match Pattern(string=w1853, regular expression=":") -> (before substring=w1852:string, after substring=w1851:string)  [unwired: 3 out]
                n656 = Reverse String(1:w1852) -> (0:w1849:string)
                n657 = Reverse String(1:w1851) -> (0:w1850:string)
                n658 = call <resource>:"GDSProject_GetProjects.vi"("error in (no error)"=w1867, "OpenProjectRef(True)"=FALSE) -> ("Projects"=w1859:string[], "error out"=w1861:errorcluster)  [unwired: 1 in, 15 out]
                n659 = case shown="\"WholeProject\"" w1856 {
                  tunnel: w1871 -> [w1875 w1879 w1883]
                  tunnel: [w1874 w1878 w1882] -> w1870
                  tunnel: w1856 -> [w1873 _ _]
                  tunnel: w1850 -> [_ w1876 w1880]
                  frame "WholeProject" {
                    n660 = Bundle By Name(cluster=w1875, "Action"=w1873, "state"=UMLEditor_statesType."ClassReversedEngineering") -> (w1874:T5)
                  }
                  frame Default {
                    n661 = Bundle By Name(cluster=w1879, "Action"=w1876, "state"=UMLEditor_statesType."ClassReversedEngineering") -> (w1878:T5)
                  }
                  frame "VI" {
                    n662 = Bundle By Name(cluster=w1883, "Action"=w1880, "state"=UMLEditor_statesType."AddNodeFromProjectTree+SyncAll") -> (w1882:T5)
                  }
                }
                n663 = Search 1D Array(1D array=w1859, element=w1863) -> (index of element=w1858:i32)  [unwired: 1 out]
                n664 = case shown="0, Default" w1858 {
                  selector: w1858 -> [w1884 _]
                  tunnel: [w1884 0 ("t")] -> w1857
                  frame 0, Default {
                  }
                  frame -1 {
                  }
                }
                n665 = Index Array(array=w1859, index=w1857) -> (element=w1862:string)
                n666 = Empty Array?(array=w1859) -> (empty?=w1860:bool)
                n667 = property on="Project" class="Ring (strict)"("Strings []"=w1859, "Value"=w1857) -> ()  [unwired: 2 in, 2 out]
                n668 = case shown="True" w1860 {
                  tunnel: w1862 -> [w1893 _]
                  tunnel: w1861 -> [w1894 w1900]
                  tunnel: [w1892 w1900] -> w1866
                  tunnel: w1849 -> [w1889 _]
                  frame False {
                    n669 = call <resource>:"UMLEditor_TargetDialog.vi"("error in (no error)"=w1894, "Target"=w1889, "GetProjectRefByName"=w1893) -> ("error out"=w1892:errorcluster, "ProjectFolder"=w1886:path, "TargetIndex"=w1890:u16, "Targets"=w1891:string[])  [unwired: 4 in, 1 out]
                    n670 = call <resource>:"GetRelativePathOption.vi"() -> ("UseProjectFolderAsBasePath"=w1888:bool)  [unwired: 1 in, 18 out]
                    n671 = case shown="True" w1888 {
                      tunnel: w1886 -> [_ w1896]
                      tunnel: File_StoredPathesActions."Set Path" ("Method (Get Path)") -> [_ w1895]
                      frame False {
                      }
                      frame True {
                        n672 = call <resource>:"File_ApplicationPaths.vi"("PathName"=UMLEditor_StoredPathes."ClassBasePath" ("UMLPathes"), "Path In"=w1896, "Method (Get Path)"=w1895) -> ()  [unwired: 1 in, 16 out]
                      }
                    }
                    n673 = property on="Target" class="Ring (strict)"("Strings []"=w1891, "Value"=w1890) -> ()  [unwired: 2 in, 2 out]
                  }
                  frame True {
                    n674 = property on="Target" class="Ring (strict)"("Strings []"=string[] [], "Value"=u16 0 ("icon")) -> ()  [unwired: 2 in, 2 out]
                  }
                }
              }
              frame "ShowInStateDiagram" {
                n675 = Match Pattern(string=w1922, regular expression=":") -> (after substring=w1917:string)  [unwired: 4 out]
                n676 = Match Pattern(string=w1917, regular expression=":") -> (before substring=w1916:string, after substring=w1902:string)  [unwired: 3 out]
                n677 = Reverse String(1:w1902) -> (0:w1907:string)
                n678 = Match Pattern(string=w1907, regular expression=":") -> (before substring=w1906:string, after substring=w1905:string)  [unwired: 3 out]
                n679 = Reverse String(1:w1906) -> (0:w1903:string)
                n680 = Reverse String(1:w1905) -> (0:w1904:string)
                n681 = call <resource>:"GDSProject_GetProjects.vi"("error in (no error)"=w1920, "OpenProjectRef(True)"=FALSE) -> ("Projects"=w1912:string[], "error out"=w1914:errorcluster)  [unwired: 1 in, 15 out]
                n682 = Search 1D Array(1D array=w1912, element=w1916) -> (index of element=w1911:i32)  [unwired: 1 out]
                n683 = case shown="-1" w1911 {
                  selector: w1911 -> [w1925 _]
                  tunnel: [w1925 0 ("t")] -> w1910
                  frame 0, Default {
                  }
                  frame -1 {
                  }
                }
                n684 = Index Array(array=w1912, index=w1910) -> (element=w1915:string)
                n685 = Empty Array?(array=w1912) -> (empty?=w1913:bool)
                n686 = property on="Project" class="Ring (strict)"("Strings []"=w1912, "Value"=w1910) -> ()  [unwired: 2 in, 2 out]
                n687 = case shown="True" w1913 {
                  tunnel: w1915 -> [w1934 _]
                  tunnel: w1914 -> [w1935 w1941]
                  tunnel: [w1933 w1941] -> w1919
                  tunnel: w1903 -> [w1930 _]
                  frame False {
                    n688 = call <resource>:"UMLEditor_TargetDialog.vi"("error in (no error)"=w1935, "Target"=w1930, "GetProjectRefByName"=w1934) -> ("error out"=w1933:errorcluster, "ProjectFolder"=w1927:path, "TargetIndex"=w1931:u16, "Targets"=w1932:string[])  [unwired: 4 in, 1 out]
                    n689 = call <resource>:"GetRelativePathOption.vi"() -> ("UseProjectFolderAsBasePath"=w1929:bool)  [unwired: 1 in, 18 out]
                    n690 = property on="Target" class="Ring (strict)"("Strings []"=w1932, "Value"=w1931) -> ()  [unwired: 2 in, 2 out]
                    n691 = case shown="True" w1929 {
                      tunnel: w1927 -> [_ w1937]
                      tunnel: File_StoredPathesActions."Set Path" ("Method (Get Path)") -> [_ w1936]
                      frame False {
                      }
                      frame True {
